vi "lab4_1.vi"() -> ()   [LabVIEW 2025]
uses:
  thresholds.ctl
  fpga_states.ctl
  <vilib>/rvi/Emulation/niFpgaGetClockAttributes.vi
  <vilib>/rvi/Emulation/niFpgaSctlEmulationGetInTimedLoop.vi
  <vilib>/rvi/Emulation/niFpgaEmulationReportErrorSimple.vi
  <vilib>/rvi/Emulation/niFpgaEmulationIsFPGAContextNoSignature.vi
  <vilib>/rvi/errors/niFpgaSetErrorForExecOnDevCompSimple.vi
  <vilib>/rvi/eio/common/nirviEmuReportErrorAndStop.vi
  <vilib>/rvi/DataTransferAndStorage/Container/Common/niFpgaContainerGetUniqueNameForEmu.vi
  <vilib>/rvi/FIFO/Fifo_Resource/nirvififoEmulationSetSize.vi
  <vilib>/rvi/FIFO/Fifo_Resource/nirviFifoEmulationQueueMgr.vi
  <instcachedir>/0/nirviFifoEmulationQueueMgr_E5CAEC123FF24DC58D834DCA3CDAA9B5.lvgen/nirviFifoEmulationQueueMgr_E5CAEC123FF24DC58D834DCA3CDAA9B5_002.vi
  <vilib>/Utility/error.llb/Clear Errors.vi
  <vilib>/rvi/FIFO/Fifo_Resource/nirvififoEmulationCreateLock.vi
  <vilib>/rvi/Emulation/niFpgaProcessEmulError.vi
  <vilib>/rvi/FIFO/Fifo_Resource/nirvififoEmulationObtainLock.vi
  <vilib>/rvi/FIFO/Fifo_Resource/nirvififoEmulationReleaseLock.vi
  <vilib>/rvi/occurrence/nirviWaitOnOccurrenceBase.vi
  <vilib>/rvi/errors/nirviReportUnexpectedCaseInternalError.vi
  <vilib>/rvi/errors/nirviReportUnexpectedCaseInternalError (U32).vi
  <vilib>/eio/utilities/niEioResolveVilibRelativePath.vi
  <vilib>/rvi/interface/RandomDataEmulation/niFpgaRandomDataHandleErrors.vi
  <vilib>/rvi/Emulation/niFpgaCriticalErrorInLSC.vi
  <vilib>/rvi/Memory/Memory_Emulation/nirvimemoryFastEmulation.vi
  <vilib>/rvi/Memory/Memory_Emulation/nirvimemoryEmulation.vi
  <vilib>/rvi/DataTransferAndStorage/Container/Common/niFpgaContainerExecOnDevCompGetState.vi
  <vilib>/rvi/Memory/Memory_Emulation/niFpgaMemoryEmulationCacheClearOnFirstRun.vi
  <vilib>/rvi/Memory/Memory_Emulation/nirvimemoryEmulationManagerCache_MakeExclusive.vi
  <vilib>/rvi/Memory/Memory_Emulation/niFpgaMemoryEmulationValidateCache.vi
  <vilib>/rvi/Memory/Memory_Emulation/nirvimemoryEmulationManagerCache_InsertValue.vi
  <vilib>/rvi/Memory/Memory_Emulation/nirvimemoryEmulationManagerCache_ReleaseExclusive.vi
  <vilib>/rvi/Memory/Memory_Emulation/nirvimemoryEmulationManagerCache_GetValue.vi
  <vilib>/rvi/Memory/Memory_Emulation/nirvimemoryEmulationManagerCache_SetValue.vi
  <vilib>/rvi/Emulation/niFpgaSctlEmulationResourceMgr.vi
  <vilib>/rvi/FIFO/Fifo_Resource/nirvififoEmulationDetermineInputValidOut.vi
  <vilib>/rvi/DataTransferAndStorage/Container/XNode/niFpgaContainer.xnode
  <vilib>/rvi/FIFO/Fifo_Resource/nirvififoEmulationRead.vi
  <vilib>/rvi/interface/RandomDataEmulation/nirviRandomDataFpgaReadWriteTemplate.vi
  <vilib>/eio/EIONode/EIONode.xnode
  <vilib>/rvi/Memory/Memory_Emulation/niFpgaMemoryEmulationRefIn.vi
  <vilib>/rvi/FIFO/Fifo_Resource/nirvififoEmulationWrite.vi
  <vilib>/rvi/eio/common/nirviEmuTemplateMethod_errors.vi
panel:
  in  "manual trigger":bool
  in  "Threshold":T1
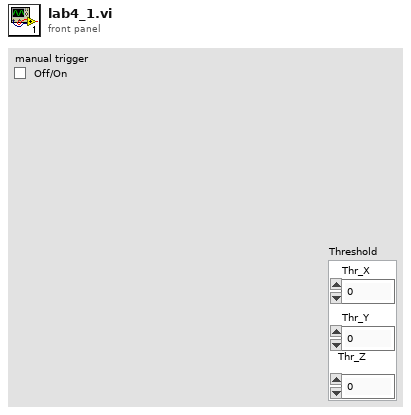
[diagram p1: front panel]
types:
  T1 = typedef "thresholds.ctl" = cluster{"Thr_X":i16, "Thr_Y":i16, "Thr_Z":i16}
  T2 = typedef "fpga_states.ctl" = enum16{"Wait", "Collect"}
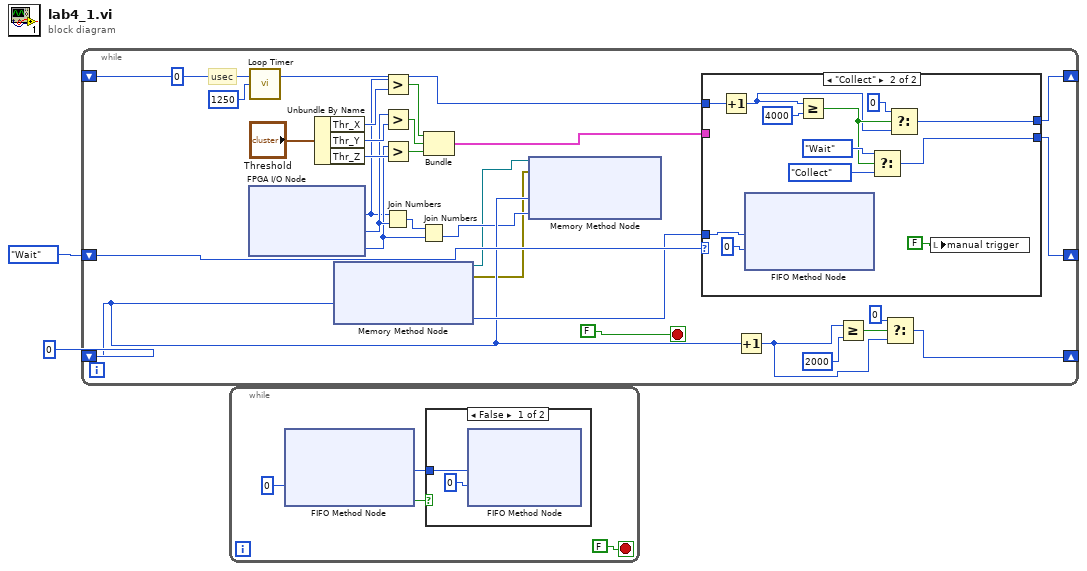
[diagram p0: block diagram]
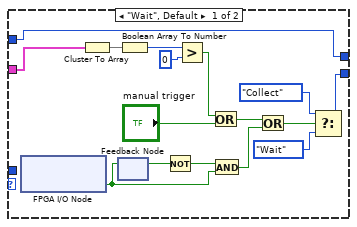
[diagram p3: hidden frame]
diagram:
  n1 = while {
    shift-right: [w28] -> _
    shift-left: i16 0 -> [w29]
    shift-right: [w18] -> _
    shift-left: fpga_states."Wait" -> [w19]
    shift-right: [w9] -> _
    shift-left: u32 0 -> [w7]
    stop <- FALSE stop-if-true
    # "usec"
    n2 = xnode "FPGA I/O Node"() -> ("AccelerationX"=w14:i16, "AccelerationY"=w16:i16, "AccelerationZ"=w15:i16)  [unwired: 3 in, 3 out]
    n3 = call "Loop Timer"("Count(uSec)"=u32 1250) -> ()  [unwired: 1 out]
    n4 = Unbundle By Name("Threshold") -> ("Thr_X"=w26:i16, "Thr_Y"=w25:i16, "Thr_Z"=w24:i16)
    n5 = xnode ("Memory Method Node")("Address"=w7) -> ("Data"=w8:u64, "error out"=w4:errorcluster, "Memory Out"=w5:refnum<k21>)  [unwired: 2 in]
    n6 = Greater?(x=w14, y=w26) -> (0:w23:bool)
    n7 = Greater?(x=w16, y=w25) -> (0:w22:bool)
    n8 = Greater?(x=w15, y=w24) -> (0:w21:bool)
    n9 = Join Numbers(hi=w14, lo=w16) -> ((hi.lo)=w17:u32)
    n10 = Join Numbers(hi=w17, lo=w15) -> ((hi.lo)=w6:u64)
    n11 = Bundle(w23, w22, w21) -> (w20:cluster{bool, bool, bool})  [unwired: 1 in]
    n12 = xnode ("Memory Method Node")("Address"=w7, "Data"=w6, "error in (no error)"=w4, "Memory In"=w5) -> ()  [unwired: 2 out]
    n13 = case shown="\"Collect\"" w19 {
      tunnel: w29 -> [w45 w52]
      tunnel: [w45 w51] -> w28
      tunnel: w20 -> [w47 _]
      tunnel: [w40 w50] -> w18
      tunnel: w8 -> [_ w49]
      frame "Wait", Default {
        n14 = xnode "FPGA I/O Node"() -> ("Button0"=w35:bool)  [unwired: 1 in, 1 out]
        n15 = Cluster To Array(cluster=w47) -> (array=w46:bool[])
        n16 = feedback-in #1(w35) -> ()
        n17 = feedback #1() -> (w33:bool)  [unwired: 1 in]
        n18 = Boolean Array To Number(Boolean array=w46) -> (number=w44:u8)
        n19 = Not(x=w33) -> (.not. x?=w34:bool)
        n20 = Greater?(x=w44, y=u8 0) -> (0:w39:bool)
        n21 = Or(x=w39, y="manual trigger") -> (x .or. y?=w38:bool)
        n22 = And(x=w34, y=w35) -> (x .and. y?=w32:bool)
        n23 = Or(x=w38, y=w32) -> (x .or. y?=w36:bool)
        n24 = Select(t=fpga_states."Collect", s=w36, f=fpga_states."Wait") -> (s? t:f=w40:T2)
      }
      frame "Collect" {
        n25 = Increment(x=w52) -> (x+1=w54:i16)
        n26 = xnode ("FIFO Method Node")("Element"=w49, "Timeout"=0) -> ()  [unwired: 1 in, 2 out]
        n27 = Greater Or Equal?(x=w54, y=i16 4000) -> (x >= y?=w55:bool)
        n28 = Select(t=fpga_states."Wait", s=w55, f=fpga_states."Collect") -> (s? t:f=w50:T2)
        n29 = Select(t=i16 0, s=w55, f=w54) -> (s? t:f=w51:i16)
        n30 = local write "manual trigger"(FALSE ("manual trigger")) -> ()
      }
    }
    n31 = Increment(x=w7) -> (x+1=w11:u32)
    n32 = Greater Or Equal?(x=w11, y=u32 2000) -> (x >= y?=w12:bool)
    n33 = Select(t=u32 0, s=w12, f=w11) -> (s? t:f=w9:u32)
  }
  n34 = while {
    stop <- FALSE stop-if-true
    n35 = xnode ("FIFO Method Node")("Timeout"=0) -> ("Element"=w62:u64, "Timed Out?"=w63:bool)  [unwired: 1 in, 1 out]
    n36 = case shown="False" w63 {
      tunnel: w62 -> [w64 _]
      frame False {
        n37 = xnode ("FIFO Method Node")("Element"=w64, "Timeout"=0) -> ()  [unwired: 1 in, 2 out]
      }
      frame True {
      }
    }
  }
